vi "Registration Complete.vi"(8 "error in (no error)":errorcluster, 11 "EventHandler":refnum<class "IEventHandler.lvclass">) -> (0 "error out":errorcluster, 3 "EventHandler":refnum<class "IEventHandler.lvclass">)   [LabVIEW 2018, in "MVA Framework.lvlib" / "ActorEvents.lvlib" / "IEventHandler.lvclass"]
doc: "注册完成"
uses:
  IEventHandler.lvclass
  <vilib>/ActorFramework/Actor/Actor.lvclass
  <vilib>/ActorFramework/Stop Msg/Stop Msg.lvclass
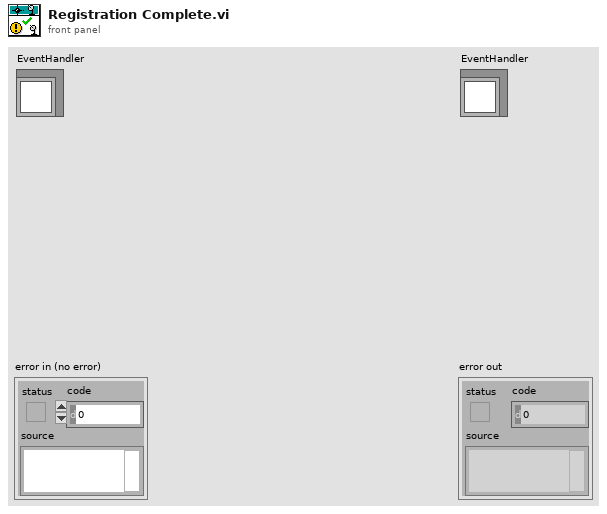
[diagram p1: front panel]
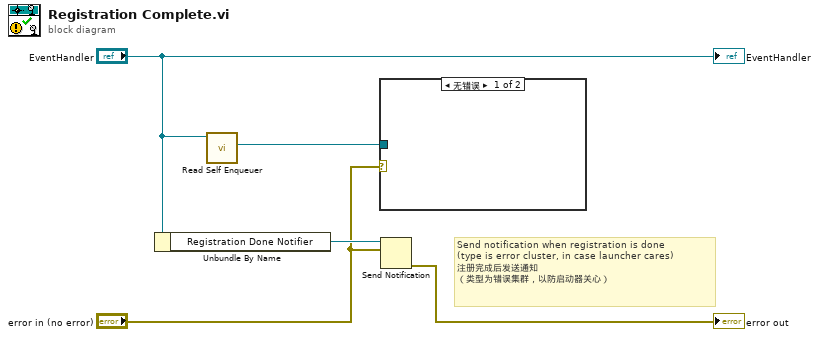
[diagram p0: block diagram]
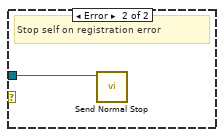
[diagram p2: hidden frame]
diagram:
  # "Send notification when registration is done\n(type is error cluster, in case launcher cares)\n注册完成后发送通知\n（类型为错误集群，以防启动器关心）"
  n1 = Unbundle By Name("EventHandler") -> ("Registration Done Notifier"=w5:refnum<notifier>)
  n2 = call <vilib>:"Read Self Enqueuer.vi"("Actor"="EventHandler") -> ("Self Enqueuer"=w1:refnum<class "Message Enqueuer.lvclass">)  [unwired: 10 in]
  n3 = case shown="无错误" "error in (no error)" {
    tunnel: w1 -> [_ w6]
    frame No Error {
    }
    frame Error {
      # "Stop self on registration error"
      n4 = call <vilib>:"Send Normal Stop.vi"("Message Enqueuer"=w6) -> ()  [unwired: 10 in, 1 out]
    }
  }
  n5 = Send Notification(notification="error in (no error)", notifier=w5) -> (error out=→"error out":errorcluster)  [unwired: 1 in, 1 out]
  "EventHandler" <- "EventHandler"
